vi "Call Import ESI File.vi"(7 "Select a device profile or file path":path, 8 "error in":errorcluster, 9 "Import to RT target":bool, 10 "Import to host PC":bool, 11 "Target IP Address":string) -> (0 "error out":errorcluster, 3 "result out":string[][](array[string]))   [LabVIEW 2020, in "SEECD System Explorer.lvlib"]
uses:
  SEECD System Explorer.lvlib
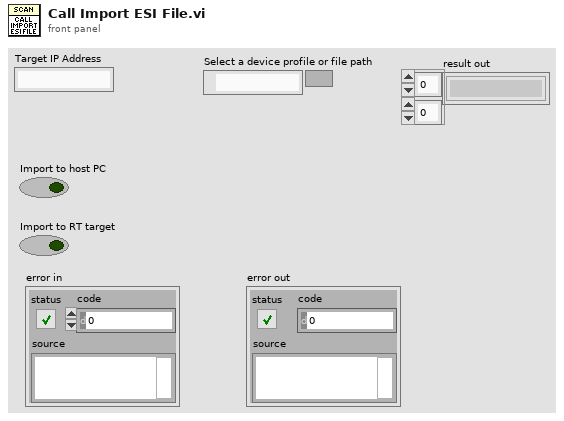
[diagram p1: front panel]
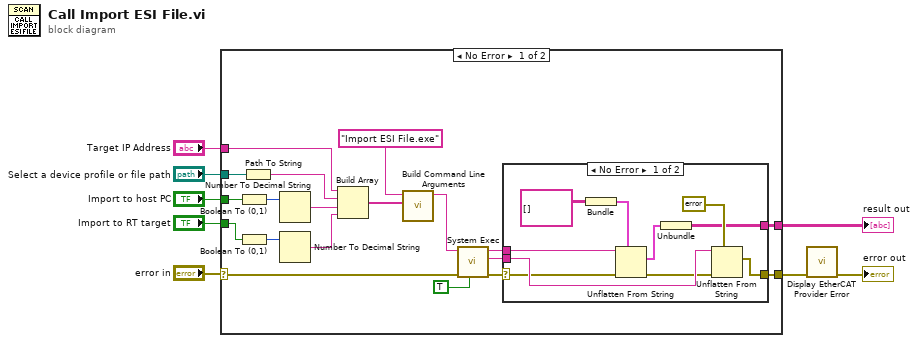
[diagram p0: block diagram]
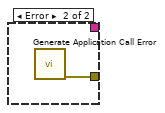
[diagram p2: hidden frame]
diagram:
  n1 = case shown="No Error" "error in" {
    selector: "error in" -> [w27 w39]
    tunnel: [w24 w39] -> w2
    tunnel: [w26 _] -> w7
    tunnel: "Import to RT target" -> [w15 _]
    tunnel: "Target IP Address" -> [w14 _]
    tunnel: "Select a device profile or file path" -> [w13 _]
    tunnel: "Import to host PC" -> [w10 _]
    frame No Error {
      n2 = Boolean To (0,1)(Boolean=w10) -> (0, 1=w11:i16)
      n3 = Boolean To (0,1)(Boolean=w15) -> (0, 1=w17:i16)
      n4 = Path To String(path=w13) -> (string=w12:string)
      n5 = Number To Decimal String(number=w11) -> (decimal integer string=w9:string)  [unwired: 1 in]
      n6 = Number To Decimal String(number=w17) -> (decimal integer string=w16:string)  [unwired: 1 in]
      n7 = Build Array(w14, w12, w9, w16) -> (w19:string[])
      n8 = call "Build Command Line Arguments.vi"("Arguments"=w19, "Executable File Name"="Import ESI File.exe" ("name or relative path")) -> ("Command Line"=w18:string)  [unwired: 9 in]
      n9 = call <vilib>:"System Exec.vi"("run minimized? (F)"=TRUE, "error in (no error)"=w27, "command line"=w18) -> ("error out"=w25:errorcluster, "standard error"=w22:string, "standard output"=w23:string)  [unwired: 5 in, 1 out]
      n10 = case shown="No Error" w25 {
        selector: w25 -> [w34 _]
        tunnel: [w30 _] -> w26
        tunnel: [w36 w38] -> w24
        tunnel: w23 -> [w33 _]
        tunnel: w22 -> [w35 _]
        frame No Error {
          n11 = Bundle("result out 2"=string[][] []) -> (w32:cluster{"result out 2":string[][]})  [unwired: 1 in]
          n12 = Unflatten From String(type=w32, binary string=w33, error in (no error)=w34) -> (value=w31:cluster{"result out 2":string[][]}, error out=w28:errorcluster)  [unwired: 2 in, 1 out]
          n13 = Unbundle(w31) -> ("result out 2"=w30:string[][])
          n14 = Unflatten From String(type=errorcluster {"status"=FALSE, "code"=0, "source"=""} ("error in (no error)"), binary string=w35, error in (no error)=w28) -> (value=w36:errorcluster)  [unwired: 2 in, 2 out]
        }
        frame Error {
          n15 = call "Generate Application Call Error.vi"() -> ("error out"=w38:errorcluster)  [unwired: 11 in]
        }
      }
    }
    frame Error {
    }
  }
  "result out" <- w7
  n16 = call "Display EtherCAT Provider Error.vi"("error in"=w2) -> ("error out"=→"error out":errorcluster)  [unwired: 10 in]
